vi "WriteQ0FileData.vi"(8 "error in (no error)":errorcluster, 10 "file data":dbl[][](array[numeric]), 11 "Scope5761 in":refnum<class "Scope5782_six_channel.lvclass">) -> (0 "error out":errorcluster, 3 "Scope5761 out":refnum<class "Scope5782_six_channel.lvclass">)   [LabVIEW 2025, in "Scope5782_six_channel.lvclass"]
uses:
  Scope5782_six_channel.lvclass
  Scope5782_six_channel.lvclass/Scope5782_six_channel.ctl
  FileStream/DumpFileAction.ctl
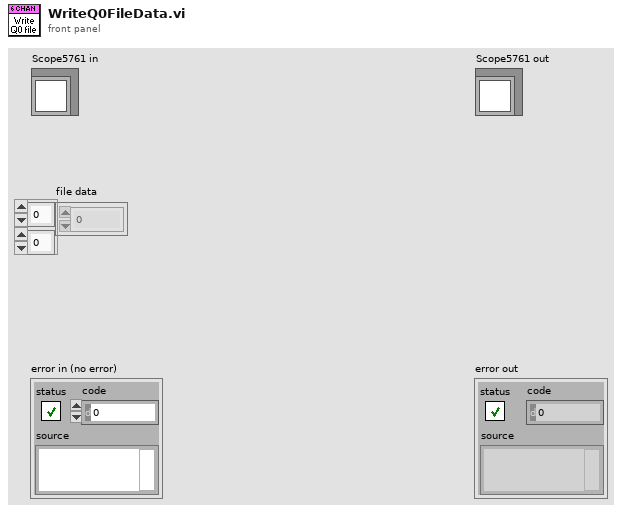
[diagram p1: front panel]
types:
  T1 = typedef "DumpFileAction.ctl" = enum16{"StartNew", "StartAppend", "Data", "Close"}
  T2 = typedef "DumpFileQueue.ctl" = refnum<queue>
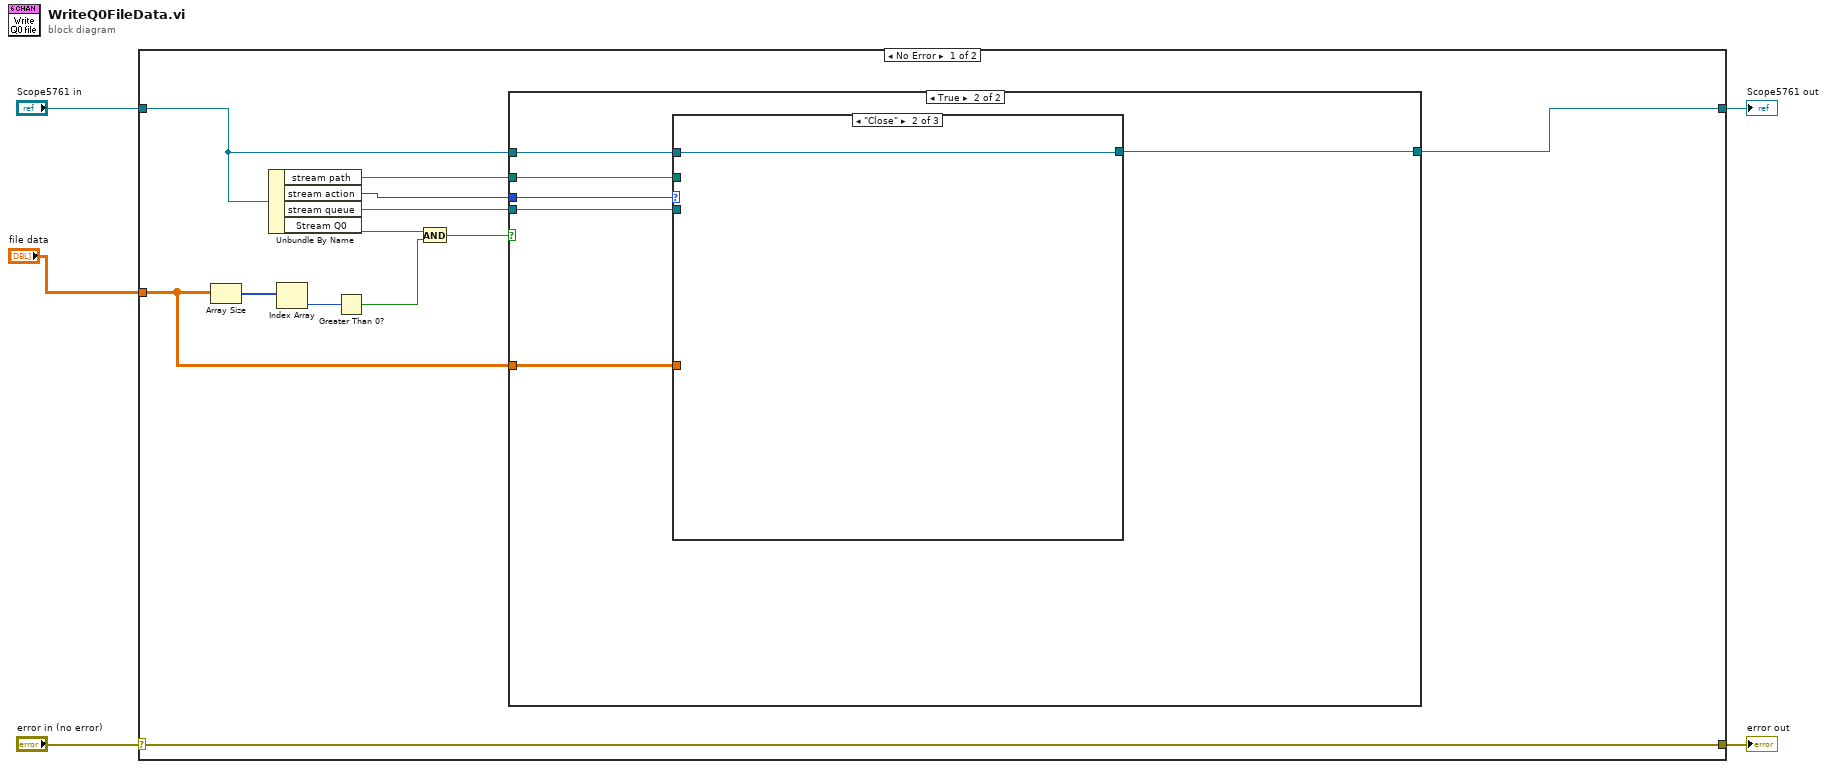
[diagram p0: block diagram]
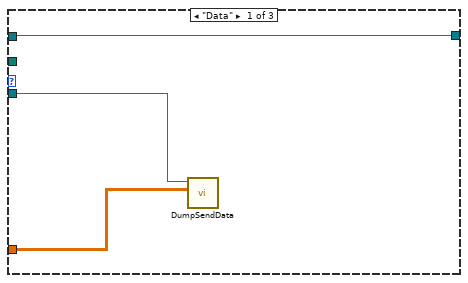
[diagram p3: hidden frame]
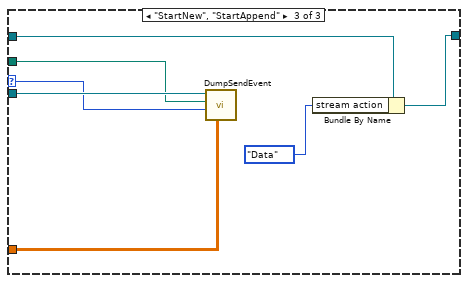
[diagram p4: hidden frame]
diagram:
  n1 = case shown="No Error" "error in (no error)" {
    selector: "error in (no error)" -> [w17 w37]
    tunnel: [w17 w37] -> w4
    tunnel: [w6 w36] -> w2
    tunnel: "Scope5761 in" -> [w7 w36]
    tunnel: "file data" -> [w11 _]
    frame No Error {
      n2 = Array Size(array=w11) -> (size(s)=w16:i32[])
      n3 = Unbundle By Name(w7) -> ("stream path"=w8:path, "stream action"=w9:T1, "stream queue"=w10:T2, "Stream Q0"=w14:bool)
      n4 = Index Array(array=w16) -> (element=w15:i32)  [unwired: 1 in]
      n5 = Greater Than 0?(x=w15) -> (x > 0?=w13:bool)
      n6 = And(x=w14, y=w13) -> (x .and. y?=w12:bool)
      n7 = case shown="True" w12 {
        tunnel: w11 -> [_ w24]
        tunnel: w10 -> [_ w23]
        tunnel: w9 -> [_ w22]
        tunnel: w8 -> [_ w21]
        tunnel: w7 -> [w18 w20]
        tunnel: [w18 w19] -> w6
        frame False {
        }
        frame True {
          n8 = case shown="\"Close\"" w22 {
            selector: w22 -> [_ _ w33]
            tunnel: w24 -> [w27 _ w32]
            tunnel: w23 -> [w26 _ w35]
            tunnel: w21 -> [_ _ w34]
            tunnel: w20 -> [w25 w28 w31]
            tunnel: [w25 w28 w29] -> w19
            frame "Data" {
              n9 = call "DumpSendData.vi"("Data"=w27, "DumpFileQueue"=w26) -> ()  [unwired: 10 in]
            }
            frame "Close" {
            }
            frame "StartNew", "StartAppend" {
              n10 = call "DumpSendEvent.vi"("Data"=w32, "DumpFileAction"=w33, "Path"=w34, "DumpFileQueue"=w35) -> ()  [unwired: 8 in]
              n11 = Bundle By Name(cluster=w31, "stream action"=DumpFileAction."Data") -> (w29:refnum<class "Scope5782_six_channel.lvclass">)
            }
          }
        }
      }
    }
    frame Error {
    }
  }
  "error out" <- w4
  "Scope5761 out" <- w2
